vi "SearchACKs(byID).vi"(8 "error in (no error)":errorcluster, 10 "ControlPacket in":refnum<class "ControlPacket.lvclass">, 11 "Session in":refnum<class "Session.lvclass">) -> (0 "error out":errorcluster, 1 "found?":bool, 2 "Pending ACK":T1 {"Packet Identifier" format="%016b"}, 3 "Session out":refnum<class "Session.lvclass">)   [LabVIEW 2013, in "MQTT Base.lvlib" / "Session.lvclass"]
uses:
  Session.lvclass
  Pending ACKs -- cluster.ctl
  <vilib>/LabVIEW Open Source Project/MQTT Control Packets/Control Packets/ControlPacket/ControlPacket.lvclass
  Session.lvclass/Session.ctl
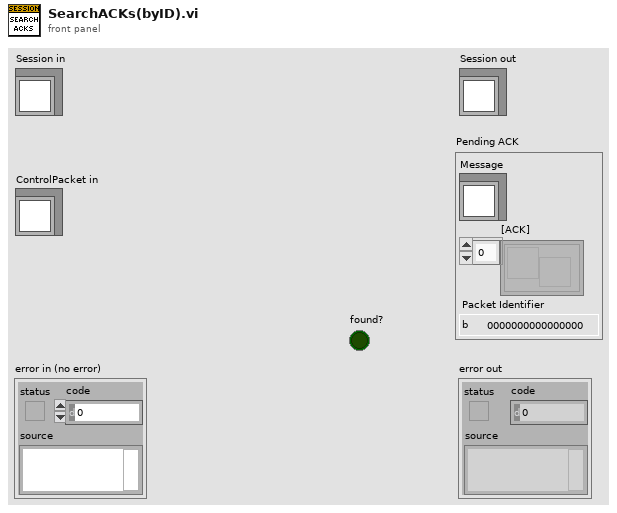
[diagram p1: front panel]
types:
  T1 = typedef "MQTT Base.lvlib/Session.lvclass/Pending ACKs -- cluster.ctl" = cluster{"Message":refnum<class "ControlPacket.lvclass">, "[ACK]":refnum<notifier>[], "Packet Identifier":u32}
  T2 = typedef "MQTT Base.lvlib/Session.lvclass/Session State -- cluster.ctl" = cluster{"CleanSession":bool, "Client ID":string, "Subscriptions":T3[], "Pending Transmissions":T5[], "Pending ACK map":variant}
  T3 = typedef "MQTT_Control_Packets.lvlib/SUBSCRIBE.lvclass/Topic Subscription -- cluster.ctl" = cluster{"Topic Filter":string, "QoS":T4}
  T4 = typedef "MQTT_Control_Packets.lvlib/ControlPacket.lvclass/QualityOfService -- enum.ctl" = enum16{"0 (At Most Once)", "1 (At Least Once)", "2 (Exactly Once)"}
  T5 = typedef "MQTT_Control_Packets.lvlib/ControlPacket.lvclass/Pending Transmission -- cluster.ctl" = cluster{"Message":refnum<class "ControlPacket.lvclass">, "QoS":T4, "Tx-Rx":bool}
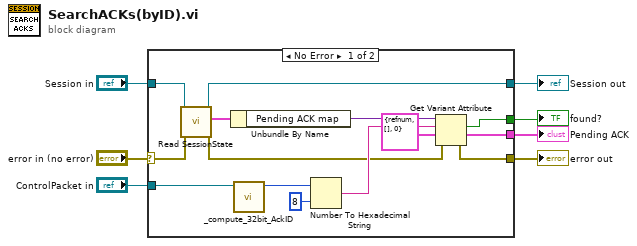
[diagram p0: block diagram]
diagram:
  n1 = case shown="No Error" "error in (no error)" {
    selector: "error in (no error)" -> [w12 w22]
    tunnel: [w13 w22] -> w6
    tunnel: [w9 w23] -> w4
    tunnel: "Session in" -> [w10 w23]
    tunnel: "ControlPacket in" -> [w20 _]
    tunnel: [w15 _] -> w2
    tunnel: [w14 _] -> w1
    frame No Error {
      n2 = call "Read SessionState.vi"("error in (no error)"=w12, "Session in"=w10) -> ("error out"=w11:errorcluster, "Session State"=w21:T2, "Session out"=w9:refnum<class "Session.lvclass">)  [unwired: 7 in]
      n3 = Unbundle By Name(w21) -> ("Pending ACK map"=w18:variant)
      n4 = call "_compute_32bit_AckID.vi"("ControlPacket in"=w20) -> ("ACK ID"=w19:u32)  [unwired: 10 in]
      n5 = Number To Hexadecimal String(1:i16 8 ("width (-)"), 2:w19) -> (0:w17:string)
      n6 = Get Variant Attribute(Variant=w18, name=w17, default value (empty Variant)=T1 {"Message"=refnum, "[ACK]"=[], "Packet Identifier"=0} ("Pending ACK"), error in=w11) -> (found=w15:bool, value=w14:T1, error out=w13:errorcluster)  [unwired: 1 out]
    }
    frame Error {
    }
  }
  "error out" <- w6
  "Session out" <- w4
  "Pending ACK" <- w1
  "found?" <- w2
